vi "Monitor_Delphi_Editor.vi"() -> ()   [LabVIEW 2015]
panel:
  out "CursorPos":cluster{"X":i32, "Y":i32}
  in  "Array":path[](array[path])=[path "C:/XctAnaDLL/Ana/Pas/KnMulti.pas", path "C:/XctAnaDLL/Ana/Pas/UTKnApp0.pas", path "C:/XctAnaDLL/Ana/Pas/TMenuApp.pas", path "C:/XctAnaDLL/Common/Pas/TKeyApp.pas", path "C:/XctAnaDLL/Common/Pas/CRT.pas", path "C:/XctAnaDLL/Ana/Pas/UTKnApp.pas", path "C:/XctAnaDLL/Ana/Pas/THaloEdi.pas", path "C:/XctAnaDLL/Delphi/XCTAnalysis_DLL.dpr", path "C:/XctAnaDLL/Ana/Pas/MenuProc.pas", path "C:/XctAnaDLL/Ana/Pas/LabViewAna.pas", path "C:/XctAnaDLL/Ana/Pas/KN_Slc.pas", path "C:/XctAnaDLL/Ana/KnMultiDelphi.dpr", path "C:/XctAnaDLL/Ana/Pas/UtAna.pas"]
  in  "Log":string
  in  "stop":bool
  in  "Mode":enum16{"Wnd from Pos", "Use HWnd Pos"}(ring)
  out "hWnd Pos":u64 format="%08x"
  out "WndPos Name":string
  out "hWnd Parent":u64 format="%08x"
  in  "ScrPos":cluster{"X":i32, "Y":i32}={"X"=1800, "Y"=300}
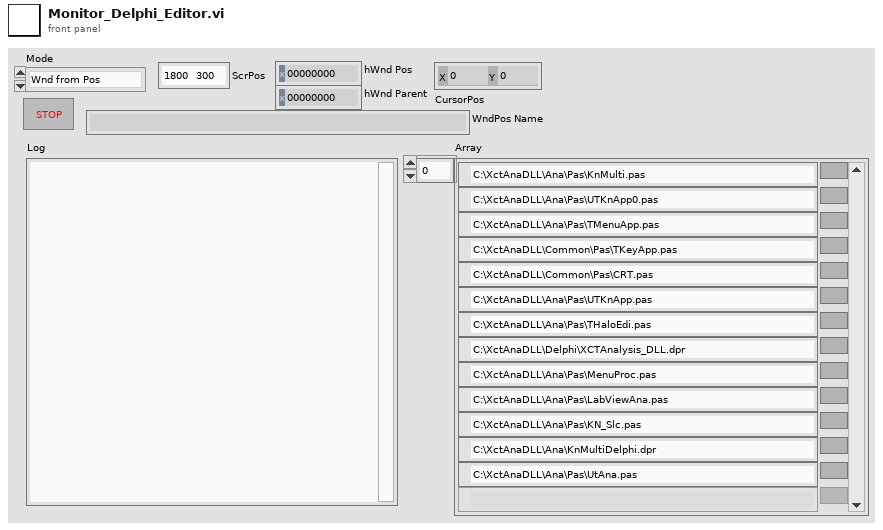
[diagram p1: front panel]
types:
  T1 = cluster{"Shift":bool, "Ctrl":bool, "Alt":bool, "Cmd":bool, "Opt":bool}
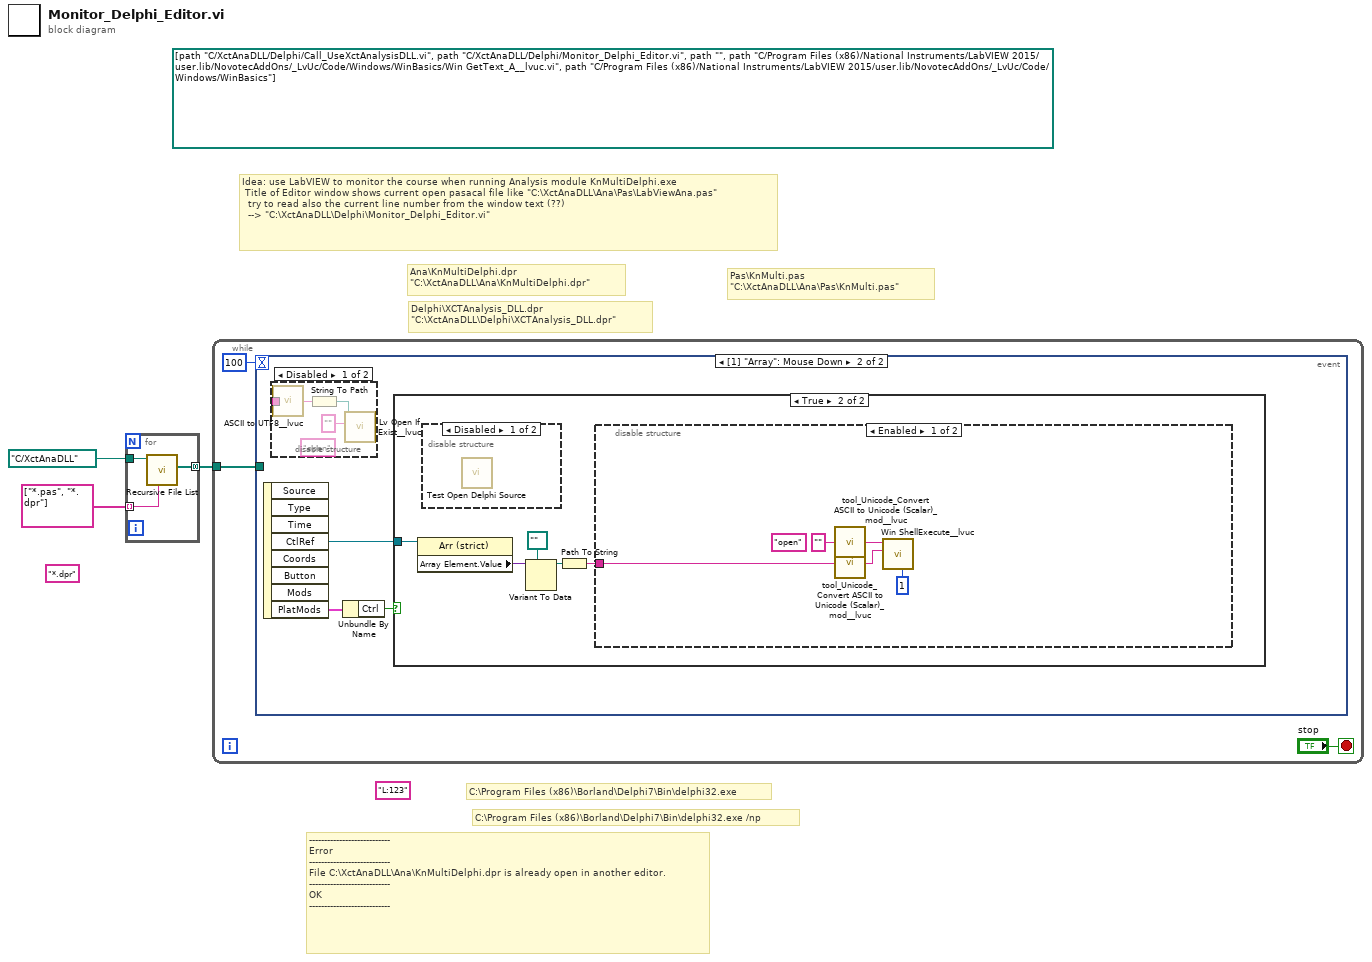
[diagram p0: block diagram]
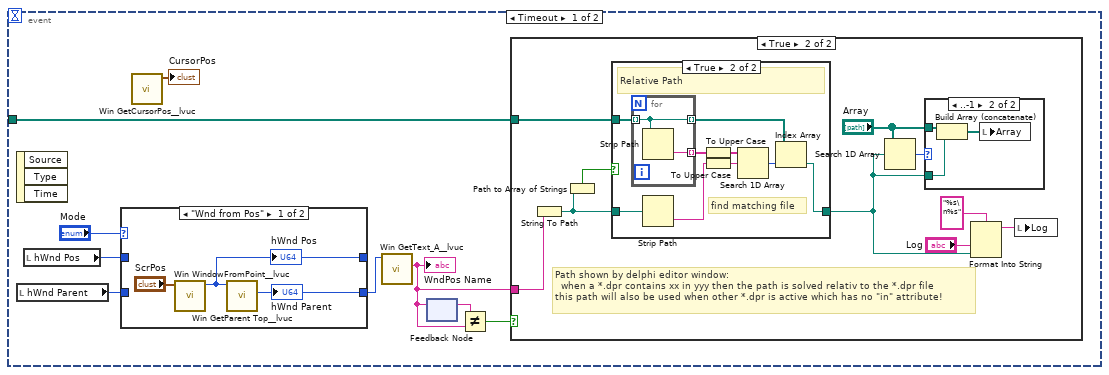
[diagram p2: hidden frame]
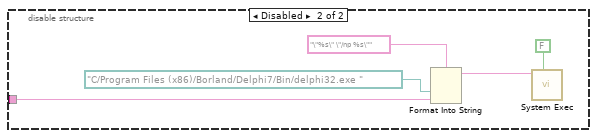
[diagram p10: hidden frame]
diagram:
  (unwired) "L:123" ("Operation (open)")
  (unwired) "*.dpr" ("pattern")
  (unwired) path[] [path "C:/XctAnaDLL/Delphi/Call_UseXctAnalysisDLL.vi", path "C:/XctAnaDLL/Delphi/Monitor_Delphi_Editor.vi", path "", path "C:/Program Files (x86)/National Instruments/LabVIEW 2015/user.lib/NovotecAddOns/_LvUc/Code/Windows/WinBasics/Win GetText_A__lvuc.vi", path "C:/Program Files (x86)/National Instruments/LabVIEW 2015/user.lib/NovotecAddOns/_LvUc/Code/Windows/WinBasics"]
  # "C:\\Program Files (x86)\\Borland\\Delphi7\\Bin\\delphi32.exe /np"
  # "C:\\Program Files (x86)\\Borland\\Delphi7\\Bin\\delphi32.exe"
  # "---------------------------\nError\n---------------------------\nFile C:\\XctAnaDLL\\Ana\\KnMultiDelphi.dpr is already open in another editor.\n---------------------------\nOK   \n---------------------------"
  # "Delphi\\XCTAnalysis_DLL.dpr\n\"C:\\XctAnaDLL\\Delphi\\XCTAnalysis_DLL.dpr\""
  # "Pas\\KnMulti.pas\n\"C:\\XctAnaDLL\\Ana\\Pas\\KnMulti.pas\""
  # "Ana\\KnMultiDelphi.dpr\n\"C:\\XctAnaDLL\\Ana\\KnMultiDelphi.dpr\""
  # "Idea: use LabVIEW to monitor the course when running Analysis module KnMultiDelphi.exe\n\tTitle of Editor window shows current open pasacal file like \"C:\\XctAnaDLL\\Ana\\Pas\\LabViewAna.pas\"\n\t\ttry to read also the current line number from the window text (??)\n\t\t--> \"C:\\XctAnaDLL\\Delphi\\Monitor_Delphi_Editor.vi\""
  n1 = for {
    tunnel: path "C:/XctAnaDLL" ("path") -> [w6]
    tunnel: string[] ["*.pas", "*.dpr"] ("pattern") -> [w5] mode=indexing
    tunnel: [w4] -> w1 mode=concatenating
    n2 = call <vilib>:"Recursive File List.vi"("pattern"=w5, "Folder Path"=w6) -> ("All Files in Dir"=w4:path[])  [unwired: 5 in, 4 out]
  }
  n3 = while {
    tunnel: w1 -> [w7]
    stop <- "stop" stop-if-true
    n4 = event shown="[1] \"Array\": Mouse Down" {
      selector: _ -> [_ _]
      dyn-events: _ -> [_ _]
      timeout: 100 -> [_ _]
      tunnel: w7 -> [w11 _]
      event Timeout {
        n5 = event-data() -> ()  [unwired: 1 in, 3 out]
        n6 = local read "hWnd Parent"() -> (w12:u64)
        n7 = local read "hWnd Pos"() -> (w17:u64)
        n8 = case shown="\"Wnd from Pos\"" "Mode" {
          tunnel: w17 -> [_ w23]
          tunnel: [w20 w23] -> _
          tunnel: [w19 w22] -> w13
          tunnel: w12 -> [_ w22]
          frame "Wnd from Pos" {
            n9 = call <userlib>:"Win WindowFromPoint__lvuc.vi"("CursorPos"="ScrPos") -> ("hWnd"=w20:i32)  [unwired: 9 in, 1 out]
            "hWnd Pos" <- w20
            n10 = call <userlib>:"Win GetParent Top__lvuc.vi"("hWnd"=w20) -> ("hWndParent"=w19:i32)  [unwired: 8 in, 2 out]
            "hWnd Parent" <- w19
          }
          frame "Use HWnd Pos", Default {
          }
        }
        n11 = call <userlib>:"Win GetCursorPos__lvuc.vi"() -> ("CursorPos Scr"=→"CursorPos":cluster{"X":i32, "Y":i32})  [unwired: 10 in, 1 out]
        n12 = call <userlib>:"Win GetText_A__lvuc.vi"("hWnd"=w13) -> ("TextA"=w14:string)  [unwired: 8 in, 2 out]
        "WndPos Name" <- w14
        n13 = feedback #1() -> (w16:string)  [unwired: 1 in]
        n14 = feedback-in #1(w14) -> ()
        n15 = Not Equal?(x=w16, y=w14) -> (x != y?=w15:bool)
        n16 = case shown="True" w15 {
          tunnel: w14 -> [_ w28]
          tunnel: w11 -> [_ w26]
          frame False {
          }
          frame True {
            # "Path shown by delphi editor window:\n  when a *.dpr contains xx in yyy then the path is solved relativ to the *.dpr file\nthis path will also be used when other *.dpr is active which has no \"in\" attribute!"
            n17 = String To Path(string=w28) -> (path=w25:path)
            n18 = Path to Array of Strings(0:w25) -> (1:w27:bool)  [unwired: 1 out]
            n19 = case shown="True" w27 {
              tunnel: [w34 w37] -> w24
              tunnel: w25 -> [w34 w42]
              tunnel: w26 -> [_ w43]
              frame False {
                # "Absolute Path"
              }
              frame True {
                # "find matching file"
                # "Relative Path"
                n20 = for {
                  tunnel: w43 -> [w44] mode=indexing
                  tunnel: [w45] -> w41 mode=indexing
                  tunnel: [w44] -> w38 mode=indexing
                  n21 = Strip Path(path=w44) -> (name=w45:string)  [unwired: 1 out]
                }
                n22 = Strip Path(path=w42) -> (name=w40:string)  [unwired: 1 out]
                n23 = To Upper Case(1:w41) -> (0:w35:string[])
                n24 = To Upper Case(1:w40) -> (0:w36:string)
                n25 = Search 1D Array(1D array=w35, element=w36) -> (index of element=w39:i32)  [unwired: 1 in]
                n26 = Index Array(array=w38, index=w39) -> (element=w37:path)
              }
            }
            n27 = Search 1D Array(1D array="Array", element=w24) -> (index of element=w30:i32)  [unwired: 1 in]
            n28 = case shown="..-1" w30 {
              tunnel: "Array" -> [_ w47]
              tunnel: w24 -> [_ w48]
              frame 0, Default {
              }
              frame ..-1 {
                n29 = Build Array (concatenate)(w47, w48) -> (w46:path[])
                n30 = local write "Array"(w46) -> ()
              }
            }
            n31 = Format Into String(format string="%s\n%s", "Log", w24) -> (resulting string=w32:string)  [unwired: 2 in, 1 out]
            n32 = local write "Log"(w32) -> ()
          }
        }
      }
      event "Array": Mouse Down {
        n33 = event-data() -> ("CtlRef"=w51:refnum<vi>, "PlatMods"=w50:T1)  [unwired: 1 in, 6 out]
        n34 = disable-structure shown="Disabled" {
          disable-tunnel: _ -> [w55 _]
          frame Disabled {
            (unwired) "open" ("Operation (open)")
            n35 = call <userlib>:"ASCII to UTF8__lvuc.vi"("ASCII"=w55) -> ("UTF8"=w54:string)  [unwired: 8 in]
            n36 = String To Path(string=w54) -> (path=w53:path)
            n37 = call <userlib>:"Lv Open If Exist__lvuc.vi"("Operation (open)"="", "Path"=w53) -> ()  [unwired: 9 in, 1 out]
          }
          frame Enabled {
          }
        }
        n38 = Unbundle By Name(w50) -> ("Ctrl"=w49:bool)
        n39 = case shown="True" w49 {
          tunnel: w51 -> [_ w60]
          frame False {
          }
          frame True {
            n40 = property class="Arr (strict)"(reference=w60) -> ("Array Element.Value"=w58:variant)  [unwired: 1 in, 2 out]
            n41 = disable-structure shown="Disabled" {
              frame Disabled {
                n42 = call "Test Open Delphi Source.vi"() -> ()  [unwired: 12 in]
              }
              frame Enabled {
              }
            }
            n43 = Variant To Data(type=path "" ("path"), Variant=w58) -> (data=w57:path)  [unwired: 1 in, 1 out]
            n44 = Path To String(path=w57) -> (string=w56:string)
            n45 = disable-structure shown="Enabled" {
              disable-tunnel: w56 -> [w61 w69]
              frame Enabled {
                (unwired) "open" ("Operation (open)")
                n46 = call <userlib>:"tool_Unicode_Convert ASCII to Unicode (Scalar)_mod__lvuc.vi"("ASCII"="" ("Operation (open)")) -> ("Unicode"=w64:string)  [unwired: 8 in]
                n47 = call <userlib>:"tool_Unicode_Convert ASCII to Unicode (Scalar)_mod__lvuc.vi"("ASCII"=w61) -> ("Unicode"=w65:string)  [unwired: 8 in]
                n48 = call <userlib>:"Win ShellExecute__lvuc.vi"("nShowCmd"=1, "FileW"=w65, "OperationW"=w64) -> ()  [unwired: 6 in, 3 out]
              }
              frame Disabled {
                n49 = Format Into String(format string="\"%s\" \"/np %s\"", path "C:/Program Files (x86)/Borland/Delphi7/Bin/delphi32.exe " ("path"), w69) -> (resulting string=w68:string)  [unwired: 2 in, 1 out]
                n50 = call <vilib>:"System Exec.vi"("wait until completion? (T)"=FALSE, "command line"=w68) -> ()  [unwired: 6 in, 4 out]
              }
            }
          }
        }
      }
    }
  }
